vi "Prepare Unicode for JSON text.vi"(4 "String in":string, 5 "Unicode (True)":bool=TRUE) -> (1 "String out":string)   [LabVIEW 2019, in "Language Selection.lvlib"]
doc: "- - -\nCopyright (c) 2026, Merecs Engineering GmbH"
uses:
  Language Selection.lvlib
  <vilib>/addons/Tools/Unicode/_subVIs/Convert ASCII to UTF-16LE (Scalar).vi
  <vilib>/addons/Tools/Unicode/_subVIs/Convert UTF-16LE to ASCII (Scalar).vi
  <vilib>/addons/Tools/Unicode/UI Unicode Tools.lvlib
panel:
  # "Connector Pane"
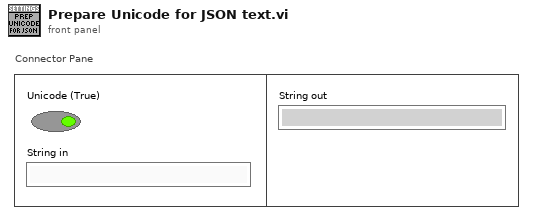
[diagram p1: front panel]
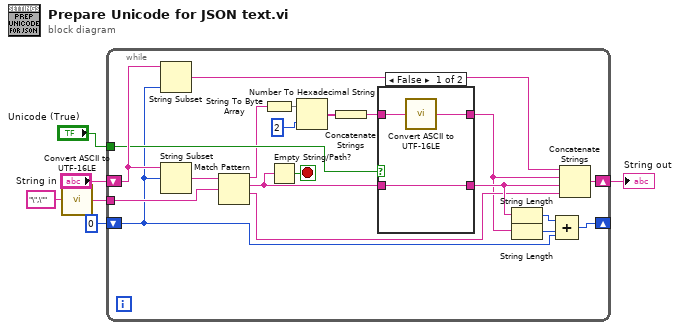
[diagram p0: block diagram]
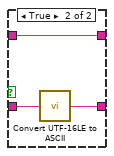
[diagram p2: hidden frame]
diagram:
  n1 = call-poly <vilib>:"Convert ASCII to UTF-16LE.vi"("ASCII"="\",\"" ("regular expression")) -> ("Unicode"=w2:string)  [unwired: 4 in]
  n2 = while {
    shift-right: [w26] -> w6
    shift-left: "String in" -> [w20]
    shift-right: [w22] -> _
    shift-left: 0 -> [w7]
    tunnel: w2 -> [w14]
    tunnel: "Unicode (True)" -> [w12]
    stop <- w25 stop-if-true
    n3 = String Subset(string=w20, length (rest)=w7) -> (substring=w21:string)  [unwired: 1 in]
    n4 = String Subset(string=w20, offset (0)=w7) -> (substring=w19:string)  [unwired: 1 in]
    n5 = Match Pattern(string=w19, regular expression=w14) -> (before substring=w8:string, match substring=w16:string, after substring=w11:string)  [unwired: 1 in, 1 out]
    n6 = String To Byte Array(string=w8) -> (unsigned byte array=w18:u8[])
    n7 = Empty String/Path?(string/path=w16) -> (empty?=w25:bool)
    n8 = Number To Hexadecimal String(1:i16 2 ("width (-)"), 2:w18) -> (0:w17:string[])
    n9 = Concatenate Strings(w17) -> (w10:string)
    n10 = case shown="False" w12 {
      tunnel: w16 -> [w29 w32]
      tunnel: [w29 w31] -> w15
      tunnel: w10 -> [w28 w30]
      tunnel: [w27 w30] -> w9
      frame False {
        n11 = call-poly <vilib>:"Convert ASCII to UTF-16LE.vi"("ASCII"=w28) -> ("Unicode"=w27:string)  [unwired: 4 in]
      }
      frame True {
        n12 = call-poly <vilib>:"Convert UTF-16LE to ASCII.vi"("Unicode"=w32) -> ("ASCII"=w31:string)  [unwired: 4 in]
      }
    }
    n13 = String Length(string=w15) -> (length=w23:i32)
    n14 = String Length(string=w9) -> (length=w24:i32)
    n15 = Compound Arithmetic op=ADD(w23, w24, w7) -> (w22:i32)
    n16 = Concatenate Strings(w21, w9, w15, w11) -> (w26:string)
  }
  "String out" <- w6
